vi "VIH Utility - STR - Match Pattern.vi"(8 "offset (0)":i32, 9 "case-sensitive (F)":bool, 10 "Regular expression":string, 11 "String":string) -> (0 "offset past match":i32, 1 "after substring":string, 2 "match substring":string, 3 "before substring":string)   [LabVIEW 2014]
doc: "::: VI Helpeks :::\nCopyright (c) 2000-2026 Konstantin Shifershteyn. All rights reserved."
panel:
  # "VI Helpeks\nCopyright (c) 2012-2026 Konstantin Shifershteyn"
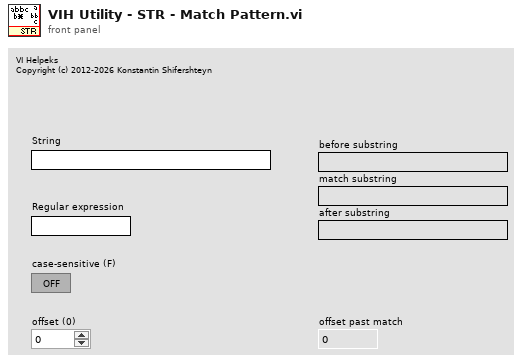
[diagram p1: front panel]
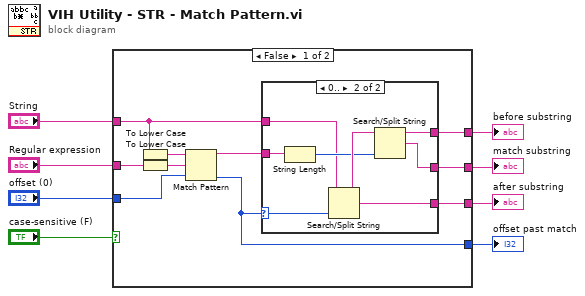
[diagram p0: block diagram]
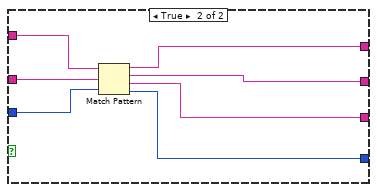
[diagram p3: hidden frame]
diagram:
  n1 = case shown="False" "case-sensitive (F)" {
    tunnel: "Regular expression" -> [w18 w34]
    tunnel: [w9 w31] -> w7
    tunnel: [w17 w30] -> w6
    tunnel: [w16 w29] -> w5
    tunnel: [w15 w28] -> w4
    tunnel: "offset (0)" -> [w14 w33]
    tunnel: "String" -> [w13 w32]
    frame False {
      n2 = To Lower Case(string=w13) -> (all lower case string=w12:string)
      n3 = To Lower Case(string=w18) -> (all lower case string=w10:string)
      n4 = Match Pattern(string=w12, regular expression=w10, offset (0)=w14) -> (before substring=w11:string, offset past match=w9:i32)  [unwired: 2 out]
      n5 = case shown="0.." w9 {
        selector: w9 -> [_ w21]
        tunnel: [w19 w22] -> w17
        tunnel: w11 -> [_ w27]
        tunnel: [_ w23] -> w16
        tunnel: [_ w24] -> w15
        tunnel: w13 -> [w19 w20]
        frame ..-1 {
        }
        frame 0.. {
          n6 = String Length(string=w27) -> (length=w25:i32)
          n7 = Search/Split String(string=w20, offset (0)=w21) -> (substring before match=w26:string, match + rest of string=w24:string)  [unwired: 1 in, 1 out]
          n8 = Search/Split String(string=w26, offset (0)=w25) -> (substring before match=w22:string, match + rest of string=w23:string)  [unwired: 1 in, 1 out]
        }
      }
    }
    frame True {
      n9 = Match Pattern(string=w32, regular expression=w34, offset (0)=w33) -> (before substring=w30:string, match substring=w29:string, after substring=w28:string, offset past match=w31:i32)
    }
  }
  "offset past match" <- w7
  "before substring" <- w6
  "match substring" <- w5
  "after substring" <- w4
